vi "Create.vi"(8 "error in":errorcluster, 10 "Parent Reference":refnum<vi>, 11 "Element in":refnum<class "Element.lvclass">) -> (0 "error out":errorcluster, 3 "Element out":refnum<class "Element.lvclass">)   [LabVIEW 2026, in "Element.lvclass"]
doc: "Create Element."
uses:
  Element.lvclass
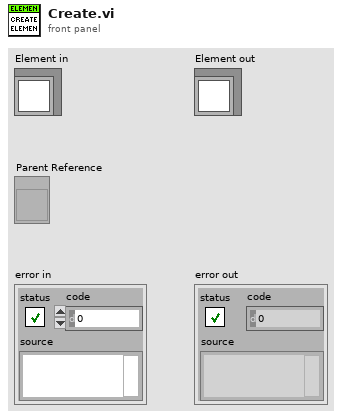
[diagram p1: front panel]
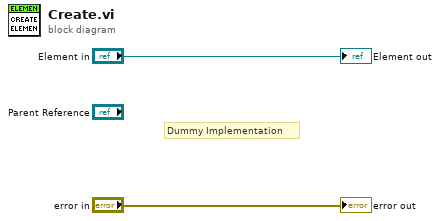
[diagram p0: block diagram]
diagram:
  # "Dummy Implementation"
  "error out" <- "error in"
  "Element out" <- "Element in"
